vi "Destroy User Events.vi"(8 "error in (no error)":errorcluster, 11 "User Events":T1) -> (0 "error out":errorcluster)   [LabVIEW 2026, in "User Event - Stop.lvlib"]
doc: "Destroy the user event, even if there is an incoming error."
uses:
  User Event - Stop.lvlib
  User Events.ctl
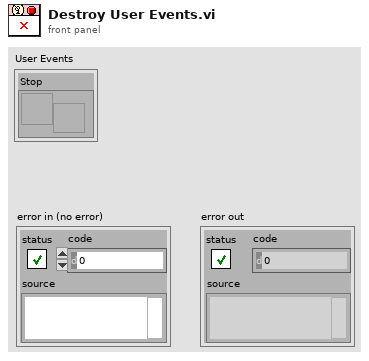
[diagram p1: front panel]
types:
  T1 = typedef "User Event - Stop.lvlib/User Events.ctl" = cluster{"Stop":refnum<user-event>}
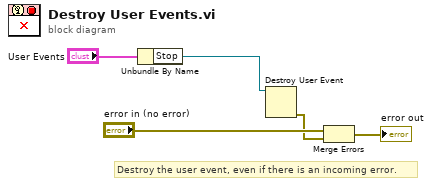
[diagram p0: block diagram]
diagram:
  # "Destroy the user event, even if there is an incoming error."
  n1 = Unbundle By Name("User Events") -> ("Stop"=w2:refnum<user-event>)
  n2 = Destroy User Event(user event=w2) -> (error out=w1:errorcluster)  [unwired: 1 in]
  n3 = Merge Errors("error in (no error)", w1) -> (→"error out":errorcluster)
